vi "Write configuration.vi"(8 "error in (no error)":errorcluster, 10 "configuration":refnum<class "CEF_serializable configuration.lvclass">, 11 "PAC in":refnum<class "PAC Instrument.lvclass">) -> (0 "error out":errorcluster, 3 "PAC out":refnum<class "PAC Instrument.lvclass">)   [LabVIEW 2025, in "PAC.lvlib" / "PAC Instrument.lvclass"]
uses:
  PAC Instrument.lvclass
  PAC Instrument.lvclass/PAC Instrument.ctl
  PAC configuration/PAC configuration.lvclass
  Users/Public/Documents/Sandia National Labs/TSS Plugin/CEF.lvlibp/serializable configuration/CEF_serializable configuration.lvclass
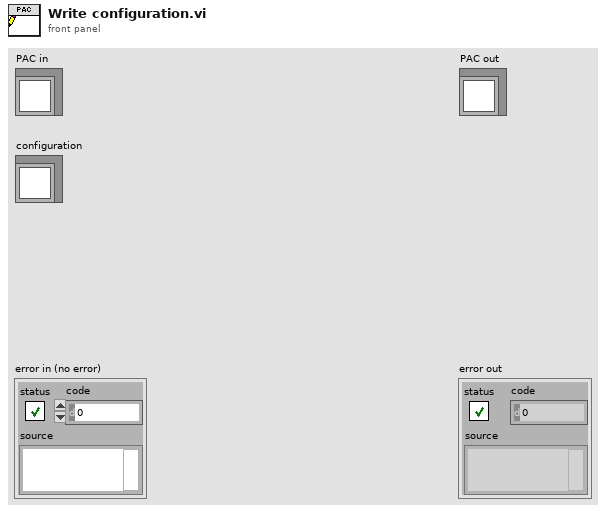
[diagram p1: front panel]
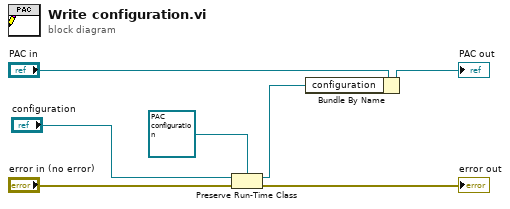
[diagram p0: block diagram]
diagram:
  n1 = Preserve Run-Time Class(object in="configuration", error in="error in (no error)", 2:refnum<class "PAC configuration.lvclass"> refnum ("PAC.lvlib:FPGA config")) -> (object out=w2:refnum<class "PAC configuration.lvclass">, error out=→"error out":errorcluster)
  n2 = Bundle By Name(cluster="PAC in", "configuration"=w2) -> (→"PAC out":refnum<class "PAC Instrument.lvclass">)
